vi "Modbus Master Test Bench.vi"(10 "Start Address":u16) -> (0 "error out":errorcluster, 2 "register values":u16[](array[numeric]))   [LabVIEW 2021]
uses:
  Modbus_RTU/Modbus_RTU.lvclass
  C:/Users/lincoln.lucio/Documents/Lincoln/Documentos Pessoais/meus docs/Projetos pessoais/Projeto Sciranda/projeto_versioned/sciranda/Modbus_Master/Modbus_Master.lvclass
  Modbus_TCP/Modbus_TCP.lvclass
  Modbus_TCP/Modbus_TCP.lvclass/Modbus_TCP.ctl
  Modbus_TCP/Accessor VIs/Write Port.vi
  Modbus_Master/Modbus_Master.lvclass
panel:
  in  "stop":bool
  in  "Combo Box":string(combo)
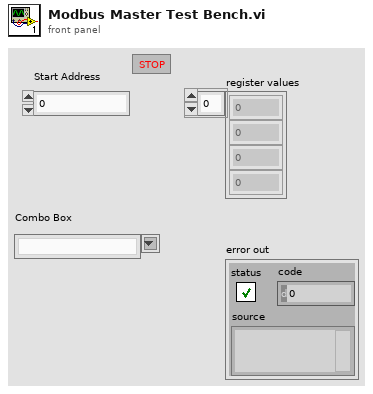
[diagram p1: front panel]
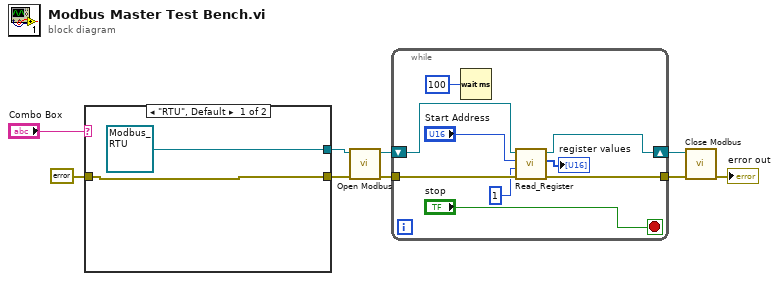
[diagram p0: block diagram]
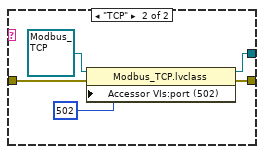
[diagram p2: hidden frame]
diagram:
  n1 = case shown="\"RTU\", Default" "Combo Box" {
    tunnel: errorcluster {"status"=FALSE, "code"=0, "source"=""} ("error in (no error)") -> [w11 w13]
    tunnel: [w11 w14] -> w3
    tunnel: [refnum<class "Modbus_RTU.lvclass"> refnum ("Modbus_RTU.lvclass") w15] -> w2
    frame "RTU", Default {
    }
    frame "TCP" {
      n2 = property class="Modbus_TCP.lvclass"(reference=refnum<class "Modbus_TCP.lvclass"> refnum ("Modbus_TCP.lvclass"), error in=w13, "Accessor VIs:port (502)"=u16 502 ("port (502)")) -> (reference out=w15:refnum<class "Modbus_TCP.lvclass">, error out=w14:errorcluster)
    }
  }
  n3 = call-dynamic "Open Modbus.vi"("error in (no error)"=w3, "Modbus_Master in"=w2) -> ("error out"=w8:errorcluster, "Modbus_Master out"=w9:refnum<class "Modbus_Master.lvclass">)  [unwired: 8 in]
  n4 = while {
    shift-right: [w22] -> w6
    shift-left: w9 -> [w25]
    tunnel: w8 -> [w24]
    tunnel: [w23] -> w7
    stop <- "stop" stop-if-true
    n5 = Wait (ms)(milliseconds to wait=u32 100) -> ()  [unwired: 1 out]
    n6 = call "Read_Register.vi"("error in (no error)"=w24, "Quantity"=u16 1, "Start Address"="Start Address", "Modbus_Master in"=w25) -> ("error out"=w23:errorcluster, "register values"=→"register values":u16[], "Modbus_Master out"=w22:refnum<class "Modbus_Master.lvclass">)  [unwired: 5 in]
  }
  n7 = call "Close Modbus.vi"("error in (no error)"=w7, "Modbus_Master in"=w6) -> ("error out"=→"error out":errorcluster)  [unwired: 8 in, 1 out]
